vi "Daily Rollup Dialog.vi"(8 "error in":errorcluster, 9 "Day Entries":T1, 10 "Day":timestamp, 11 "Project Store in":refnum<class "Project Store.lvclass">) -> (0 "error out":errorcluster, 3 "Project Store out":refnum<class "Project Store.lvclass">)   [LabVIEW 2026]
doc: "Modal dialog that shows the day's time rolled up per project and task for a timesheet (Day Rollup.vi, with Now as the current time): one row per task with Project, Task, Hours (rounded to the quarter hour, two decimals) and the joined Descriptions, plus the Total of the rounded hours.\n\nClicking a row copies that row's Descriptions to the Windows clipboard and the status line says \"Copied: Project / Task\". Copy All copies the whole table (Project TAB Task TAB Hours TAB Descriptions, rows joined by CR LF) so it pastes into a spreadsheet. Close or the window's X ends the dialog. Nothing is written to disk.\n\nInputs: Project Store in; Day (the displayed day, for the title); Day Entries (the day's entries, e.g. from Load Day.vi); error in.\nOutputs: Project Store out; error out.\n\nGenerated by: Claude"
uses:
  Storage/Project Store/Project Store.lvclass
  Storage/Rows/Time Entry List.ctl
  Storage/Rows/Time Entry.ctl
panel:
  in  "Close":bool
  in  "Copy All":bool
  in  "Roll-up":i32(listbox)
  out "Status":string
  out "Total":string
  out "Title":string
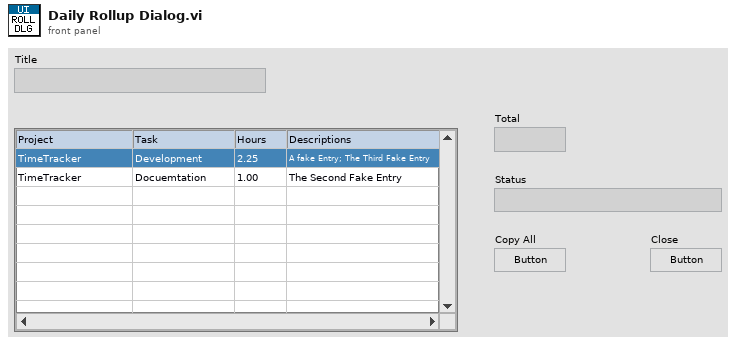
[diagram p1: front panel]
types:
  T1 = typedef "Time Entry List.ctl" = T2[]
  T2 = typedef "Time Entry.ctl" = cluster{"ID":string, "Project ID":string, "Task ID":string, "Start Time":timestamp, "End Time":timestamp, "Description":string}
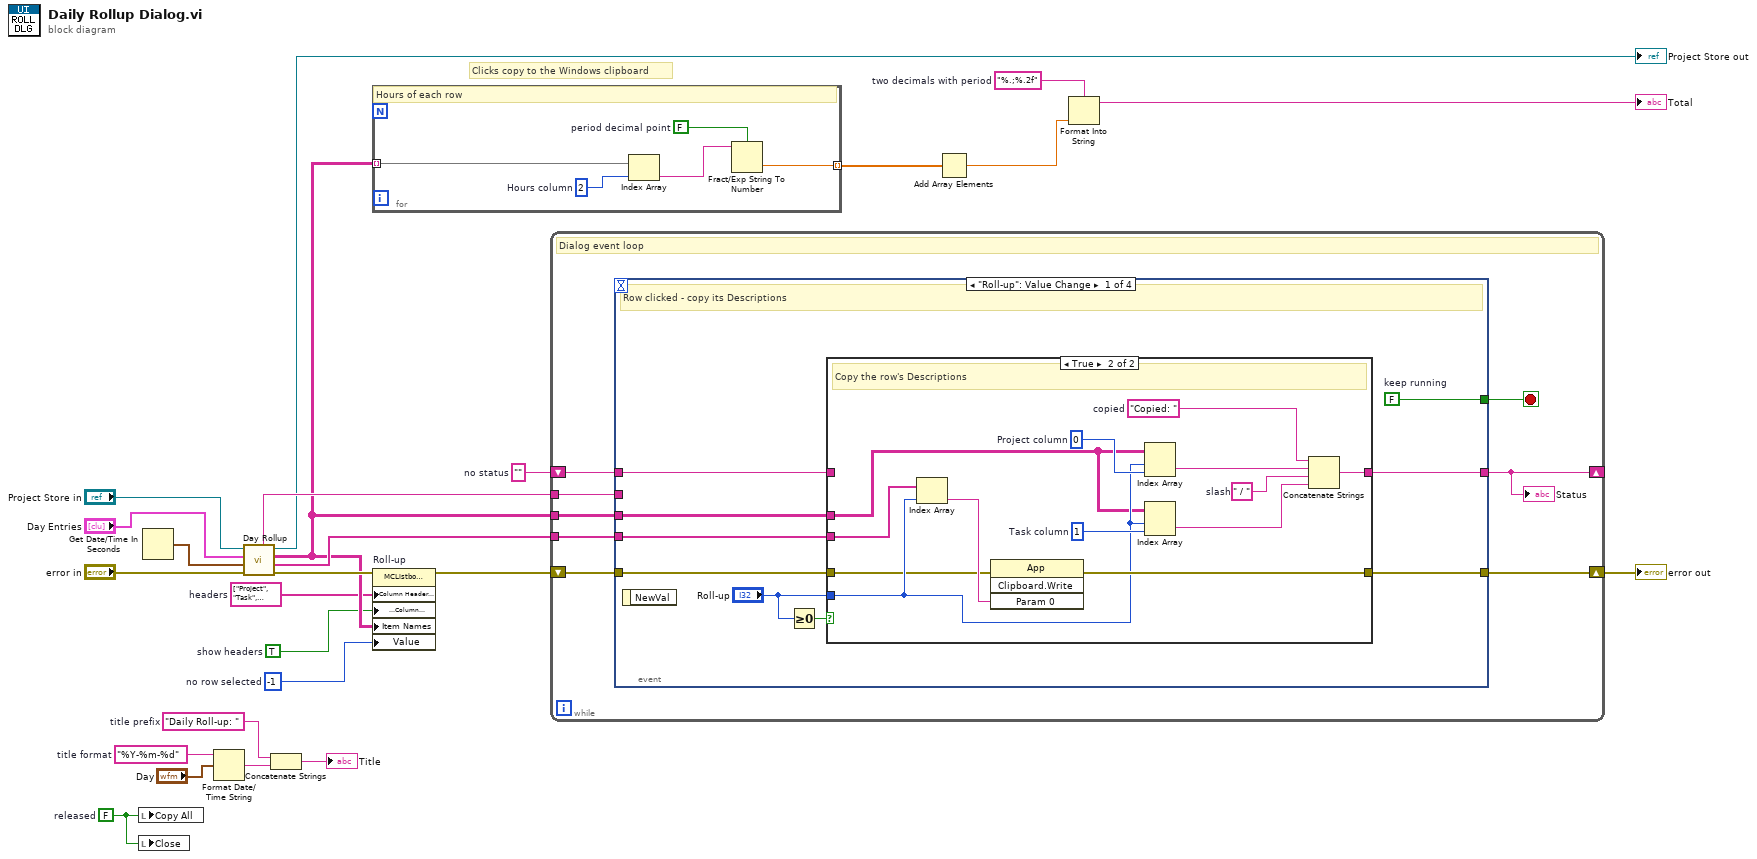
[diagram p0: block diagram]
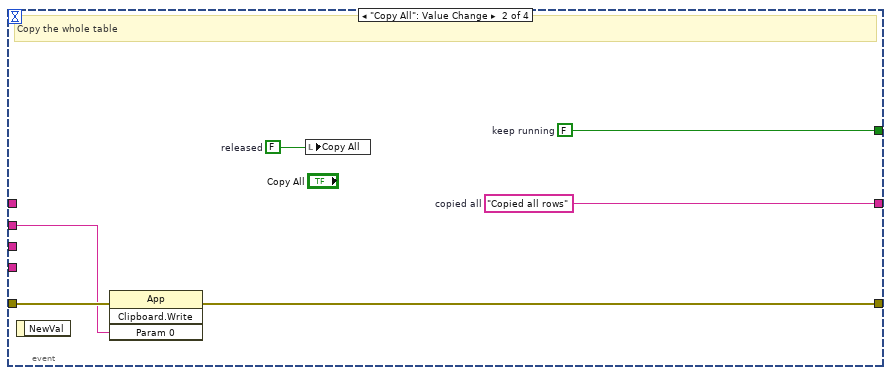
[diagram p3: hidden frame]
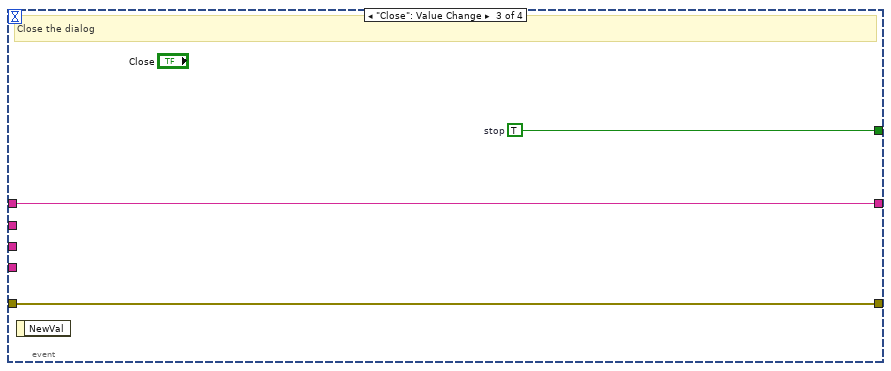
[diagram p4: hidden frame]
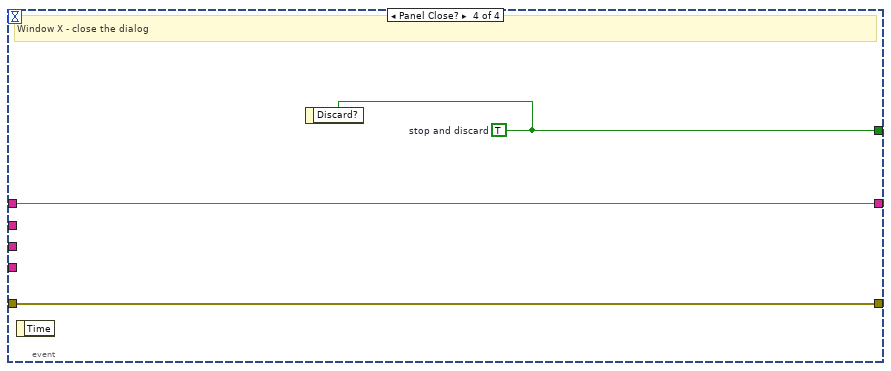
[diagram p5: hidden frame]
diagram:
  w16 = "%.;%.2f"  # two decimals with period
  w15 = ""  # no status
  w14 = FALSE  # released
  w13 = -1  # no row selected
  w12 = TRUE  # show headers
  w11 = string[] ["Project", "Task", "Hours", "Descriptions"]  # headers
  w10 = "Daily Roll-up: "  # title prefix
  w9 = "%Y-%m-%d"  # title format
  # "Clicks copy to the Windows clipboard"
  n1 = local write "Copy All"(w14) -> ()
  n2 = local write "Close"(w14) -> ()
  n3 = Get Date/Time In Seconds() -> (seconds since 1Jan1904=w17:timestamp)
  n4 = Format Date/Time String(time format string (%c)=w9, seconds (now)="Day") -> (date/time string=w22:string)  [unwired: 1 out]
  n5 = call "Day Rollup.vi"("error in"="error in", "Now"=w17, "Day Entries"="Day Entries", "Project Store in"="Project Store in") -> ("error out"=w21:errorcluster, "Row Copy Text"=w19:string[], "Rollup Rows"=w18:string[][], "Project Store out"=→"Project Store out":refnum<class "Project Store.lvclass">, "All Copy Text"=w20:string)  [unwired: 3 in]
  n6 = Concatenate Strings(w10, w22) -> (→"Title":string)
  n7 = for {
    tunnel: w18 -> [w26] mode=indexing
    tunnel: [w30] -> w24 mode=indexing
    w28 = FALSE  # period decimal point
    w27 = 2  # Hours column
    # "Hours of each row"
    n8 = Index Array(array=w26, index=w27) -> (element=w29:string)
    n9 = Fract/Exp String To Number(use system decimal point (T)=w28, string=w29) -> (number=w30:dbl)  [unwired: 2 in, 1 out]
  }
  n10 = property on="Roll-up" class="MCListbox (strict)"(error in=w21, "Column Header Strings[]"=w11, "Visible Items:Column Headers Visible"=w12, "Item Names"=w18, "Value"=w13) -> (error out=w23:errorcluster)  [unwired: 1 in, 1 out]
  n11 = while {
    shift-right: [w35] -> _
    shift-left: w15 -> [w34]
    tunnel: w18 -> [w31]
    tunnel: w19 -> [w32]
    tunnel: w20 -> [w33]
    shift-right: [w37] -> w6
    shift-left: w23 -> [w36]
    stop <- w38 stop-if-true
    # "Dialog event loop"
    n12 = event shown="[0] \"Roll-up\": Value Change" {
      selector: _ -> [_ _ _ _]
      dyn-events: _ -> [_ _ _ _]
      timeout: _ -> [_ _ _ _]
      tunnel: [w43 w65 w71 w72] -> w38
      tunnel: w34 -> [w41 _ w69 w73]
      tunnel: w31 -> [w39 _ _ _]
      tunnel: w32 -> [w40 _ _ _]
      tunnel: w33 -> [_ w63 _ _]
      tunnel: w36 -> [w42 w64 w70 w74]
      tunnel: [w44 w66 w69 w73] -> w35
      tunnel: [w45 w67 w70 w74] -> w37
      event "Roll-up": Value Change {
        w43 = FALSE  # keep running
        # "Row clicked - copy its Descriptions"
        n13 = event-data() -> ()  [unwired: 1 in, 1 out]
        n14 = Greater Or Equal To 0?(x="Roll-up") -> (x >= 0?=w47:bool)
        n15 = case shown="True" w47 {
          tunnel: "Roll-up" -> [_ w53]
          tunnel: w41 -> [w48 _]
          tunnel: [w48 w54] -> w44
          tunnel: w39 -> [_ w50]
          tunnel: w40 -> [_ w51]
          tunnel: w42 -> [w49 w52]
          tunnel: [w49 w55] -> w45
          frame False {
            # "No row - nothing to copy"
          }
          frame True {
            w59 = " / "  # slash
            w58 = "Copied: "  # copied
            w57 = 1  # Task column
            w56 = 0  # Project column
            # "Copy the row's Descriptions"
            n16 = Index Array(array=w51, index=w53) -> (element=w60:string)
            n17 = invoke class="App" method="Clipboard.Write"(error in=w52, "Param 0"=w60) -> (error out=w55:errorcluster)  [unwired: 2 in, 3 out]
            n18 = Index Array(array=w50, index (row)=w53, index (col)=w56) -> (element=w61:string)
            n19 = Index Array(array=w50, index (row)=w53, index (col)=w57) -> (element=w62:string)
            n20 = Concatenate Strings(w58, w61, w59, w62) -> (w54:string)
          }
        }
      }
      event "Copy All": Value Change {
        w68 = FALSE  # released
        w66 = "Copied all rows"  # copied all
        w65 = FALSE  # keep running
        # "Copy the whole table"
        n21 = event-data() -> ()  [unwired: 1 in, 1 out]
        n22 = invoke class="App" method="Clipboard.Write"(error in=w64, "Param 0"=w63) -> (error out=w67:errorcluster)  [unwired: 2 in, 3 out]
        n23 = local write "Copy All"(w68) -> ()
      }
      event "Close": Value Change {
        w71 = TRUE  # stop
        # "Close the dialog"
        n24 = event-data() -> ()  [unwired: 1 in, 1 out]
      }
      event Panel Close? {
        w72 = TRUE  # stop and discard
        # "Window X - close the dialog"
        n25 = event-data() -> ()  [unwired: 1 in, 1 out]
        n26 = event-data("Discard?"=w72) -> ()  [unwired: 1 in, 1 out]
      }
    }
    "Status" <- w35
  }
  "error out" <- w6
  n27 = Add Array Elements(numeric array=w24) -> (sum=w25:dbl)
  n28 = Format Into String(format string=w16, w25) -> (resulting string=→"Total":string)  [unwired: 2 in, 1 out]
